vi "RP1210 Get Last Error Msg.vi"(8 "error in (no error)":errorcluster, 10 "nClientID":i16, 11 "ErrorCode":i16) -> (0 "error out":errorcluster, 1 "function return":i16, 2 "fpchDescription":string, 3 "SubErrorCode":i32)   [LabVIEW 2020, in "cansub_rp1210.lvlib"]
doc: "short __stdcall RP1210_GetLastErrorMsg(short ErrorCode, int *SubErrorCode, char *fpchDescription,\n short nClientID);"
uses:
  cansub_rp1210.lvlib
  cansub_lv64.dll
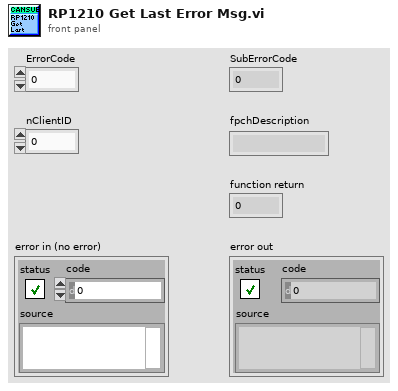
[diagram p1: front panel]
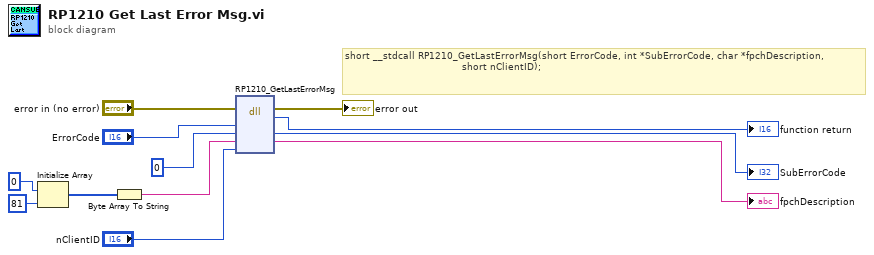
[diagram p0: block diagram]
diagram:
  # "short __stdcall RP1210_GetLastErrorMsg(short ErrorCode, int *SubErrorCode, char *fpchDescription,\n                                       short nClientID);"
  n1 = Initialize Array(u8 0 ("element"), 81 ("dimension size")) -> (w8:u8[])
  n2 = Byte Array To String(unsigned byte array=w8) -> (string=w7:string)
  n3 = dll-call lib="C:/cansub-lv/library/cansub_lv*.*" fn="RP1210_GetLastErrorMsg"(error in="error in (no error)", "ErrorCode"="ErrorCode", "SubErrorCode"=0, "fpchDescription"=w7, "nClientID"="nClientID") -> (error out=→"error out":errorcluster, "return type"=→"function return":i16, "SubErrorCode"=→"SubErrorCode":i32, "fpchDescription"=→"fpchDescription":string)  [unwired: 4 in, 1 out]
